vi "GetConnectionStatus.vi"(8 "error in (no error)":errorcluster, 11 "object in":refnum<class "DIO_Channel.lvclass">) -> (0 "error out":errorcluster, 2 "Connected?":bool, 3 "object out":refnum<class "DIO_Channel.lvclass">)   [LabVIEW 2021, in "DIO-Channel.lvlib" / "DIO_Channel.lvclass"]
uses:
  DIO_Channel.lvclass
  DIO_Channel.lvclass/DIO_Channel.ctl
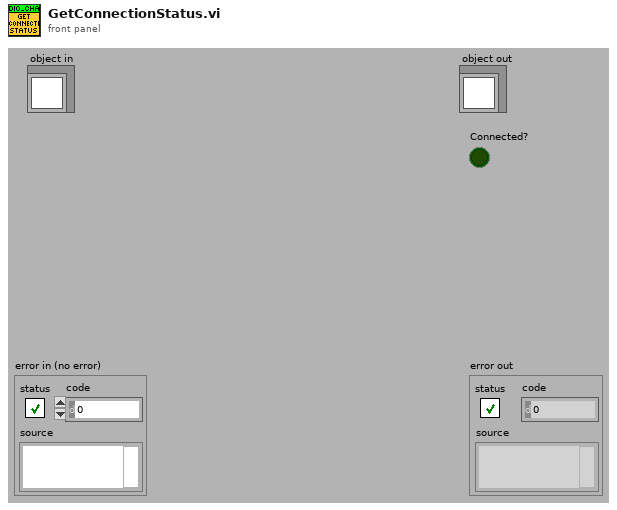
[diagram p1: front panel]
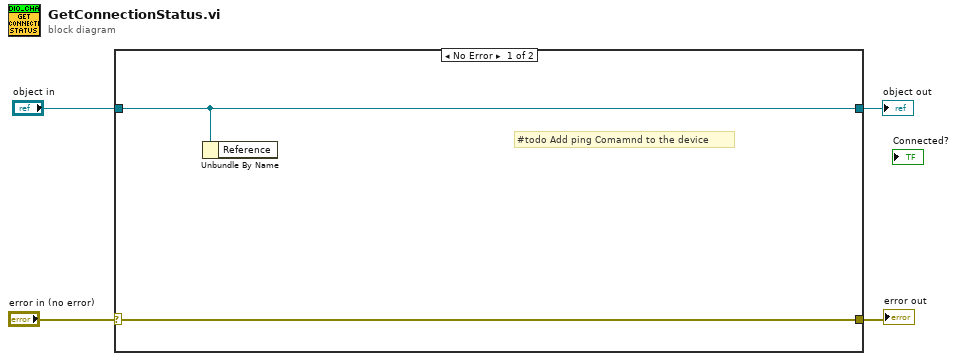
[diagram p0: block diagram]
diagram:
  n1 = case shown="No Error" "error in (no error)" {
    selector: "error in (no error)" -> [w6 w8]
    tunnel: [w6 w8] -> w3
    tunnel: [w5 w7] -> w1
    tunnel: "object in" -> [w5 w7]
    frame No Error {
      # "#todo Add ping Comamnd to the device"
      n2 = Unbundle By Name(w5) -> ()  [unwired: 1 out]
    }
    frame Error {
    }
  }
  "error out" <- w3
  "object out" <- w1
